vi "Bootstrap.vi"(8 "error in (no error)":errorcluster, 10 "Migrations Folder":path, 11 "SQLite Connection in":refnum<class "Connection.lvclass">) -> (0 "error out":errorcluster, 3 "SQLite Connection out":refnum<class "Connection.lvclass">)   [LabVIEW 2024, in "DBMigrations.lvlib"]
doc: "Apply bootstrap migration file to account for databases that haven't been versioned."
uses:
  DBMigrations.lvlib
  <vilib>/drjdpowell/SQLite Library/SQL Connection/Connection.lvclass
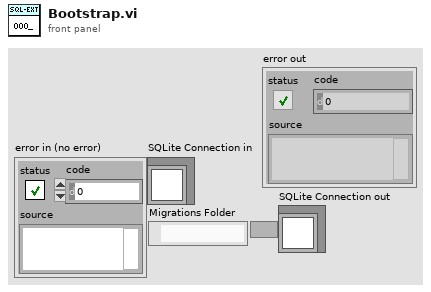
[diagram p1: front panel]
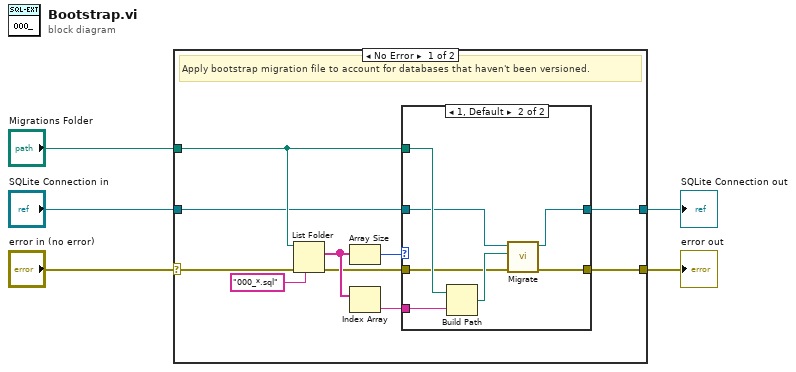
[diagram p0: block diagram]
diagram:
  n1 = case shown="No Error" "error in (no error)" {
    selector: "error in (no error)" -> [w6 w25]
    tunnel: "Migrations Folder" -> [w11 _]
    tunnel: "SQLite Connection in" -> [w10 w26]
    tunnel: [w8 w25] -> w3
    tunnel: [w7 w26] -> w2
    frame No Error {
      # "Apply bootstrap migration file to account for databases that haven't been versioned."
      n2 = List Folder(path=w11, pattern="000_*.sql", error in=w6) -> (filenames=w13:string[], error out=w9:errorcluster)  [unwired: 1 in, 2 out]
      n3 = Array Size(array=w13) -> (size(s)=w14:i32)
      n4 = Index Array(array=w13) -> (element=w12:string)  [unwired: 1 in]
      n5 = case shown="1, Default" w14 {
        tunnel: w12 -> [_ w24]
        tunnel: w11 -> [_ w23]
        tunnel: w10 -> [w17 w21]
        tunnel: w9 -> [w16 w20]
        tunnel: [w17 w19] -> w7
        tunnel: [w16 w18] -> w8
        frame 0 {
        }
        frame 1, Default {
          n6 = Build Path(base path=w23, name or relative path=w24) -> (appended path=w22:path)
          n7 = call "Migrate.vi"("error in (no error)"=w20, "Migration File Path"=w22, "SQLite Connection in"=w21) -> ("error out"=w18:errorcluster, "SQLite Connection out"=w19:refnum<class "Connection.lvclass">)  [unwired: 7 in]
        }
      }
    }
    frame Error {
    }
  }
  "error out" <- w3
  "SQLite Connection out" <- w2
